vi "Decode Frames.vi"(8 "error in":errorcluster, 10 "data in":string, 11 "pending bytes":string) -> (0 "error out":errorcluster, 2 "decoded frames":T1[](array[typedef]), 3 "remaining bytes":string)   [LabVIEW 2015, in "Lengmur_socket.lvlib"]
uses:
  Lengmur_socket.lvlib
  Types/Decoded Frame.ctl
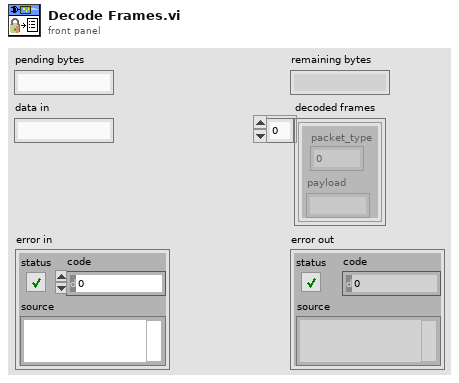
[diagram p1: front panel]
types:
  T1 = typedef "Lengmur_socket.lvlib/Decoded Frame.ctl" = cluster{"packet_type":u8, "payload":string}
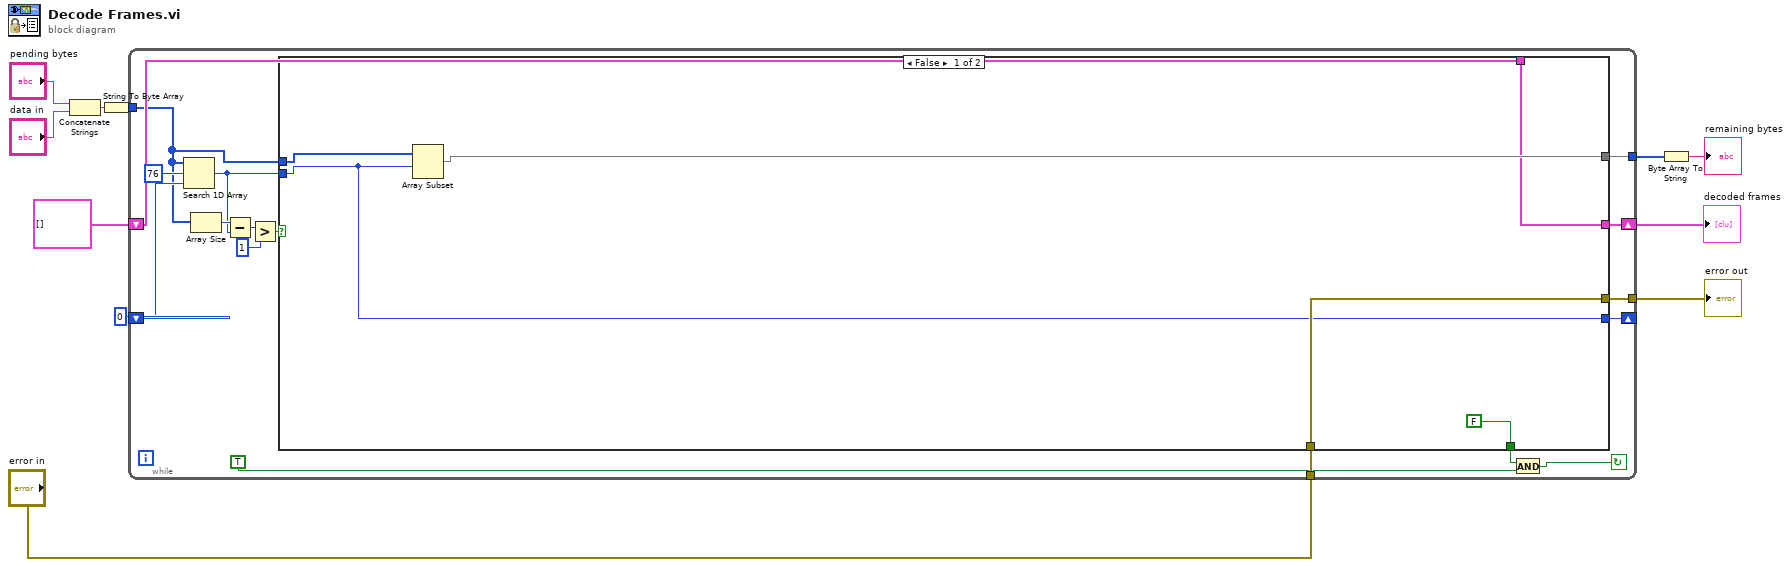
[diagram p0: block diagram]
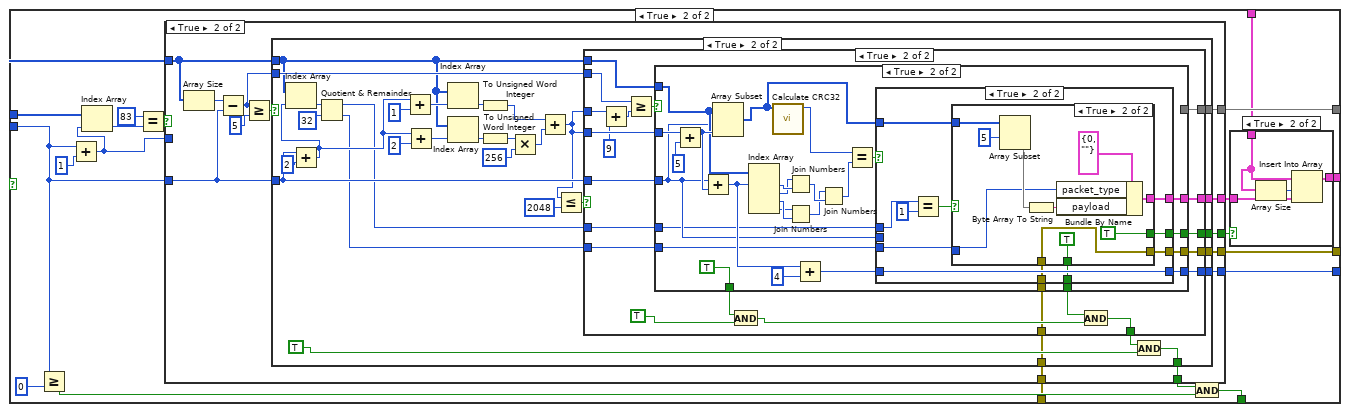
[diagram p2: hidden frame]
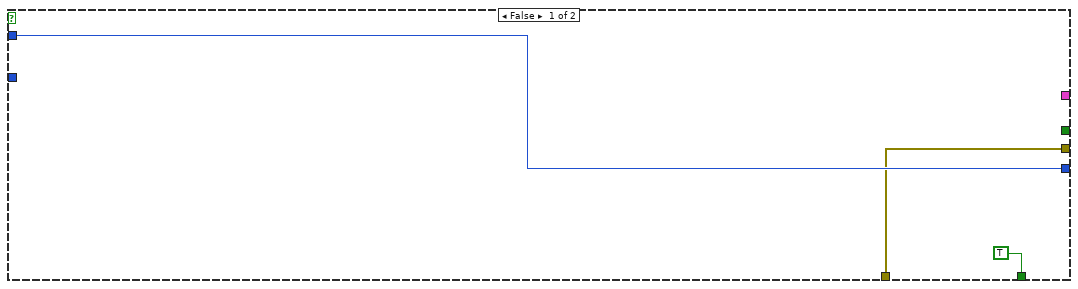
[diagram p3: hidden frame]
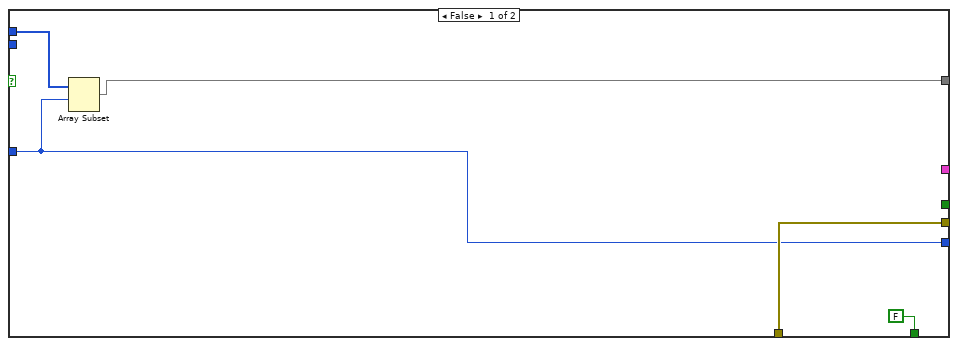
[diagram p4: hidden frame]
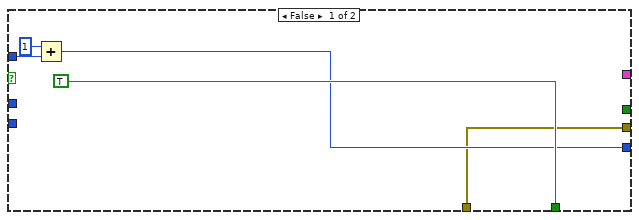
[diagram p5: hidden frame]
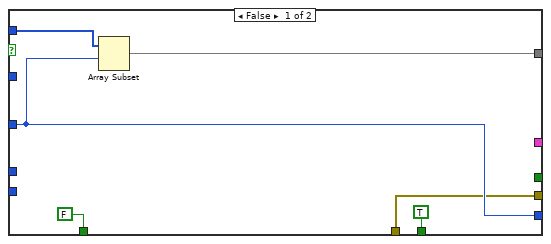
[diagram p6: hidden frame]
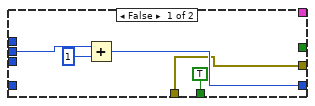
[diagram p7: hidden frame]
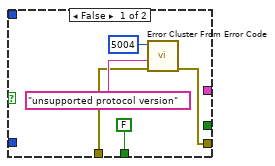
[diagram p8: hidden frame]
diagram:
  n1 = Concatenate Strings("pending bytes", "data in") -> (w9:string)
  n2 = String To Byte Array(string=w9) -> (unsigned byte array=w6:u8[])
  n3 = while {
    tunnel: w6 -> [w19]
    shift-right: [w26] -> _
    shift-left: 0 -> [w27]
    tunnel: [w25] -> w1
    tunnel: "error in" -> [w24]
    tunnel: [w23] -> w2
    shift-right: [w22] -> w4
    shift-left: T1[] [] ("decoded_frames") -> [w21]
    stop <- w13 continue-if-true
    n4 = Search 1D Array(1D array=w19, element=u8 76, start index (0)=w27) -> (index of element=w18:i32)
    n5 = Array Size(array=w19) -> (size(s)=w20:i32)
    n6 = Subtract(x=w20, y=w18) -> (x-y=w17:i32)
    n7 = Greater?(x=w17, y=1) -> (0:w15:bool)
    n8 = case shown="False" w15 {
      tunnel: [w31 w48] -> w26
      tunnel: [w33 w47] -> w25
      tunnel: w24 -> [w32 w45]
      tunnel: [w32 w44] -> w23
      tunnel: [w29 w40] -> w22
      tunnel: w21 -> [w29 w39]
      tunnel: w19 -> [w34 w37]
      tunnel: w18 -> [w31 w36]
      tunnel: [FALSE w35] -> w12
      frame False {
        n9 = Array Subset(array=w34, index=w31) -> (w33:u8[])  [unwired: 1 in]
      }
      frame True {
        n10 = Greater Or Equal?(x=w36, y=0) -> (x >= y?=w49:bool)
        n11 = Add(x=w36, y=u8 1) -> (x+y=w42:i32)
        n12 = Index Array(array=w37, index=w42) -> (element=w43:u8)
        n13 = Equal?(x=u8 83, y=w43) -> (x = y?=w52:bool)
        n14 = case shown="True" w52 {
          tunnel: [w56 w60] -> w48
          tunnel: w42 -> [w56 _]
          tunnel: w37 -> [_ w65]
          tunnel: w36 -> [_ w61]
          tunnel: [_ w66] -> w47
          tunnel: [TRUE w64] -> w46
          tunnel: w45 -> [w54 w63]
          tunnel: [w54 w62] -> w44
          tunnel: [_ w58] -> w41
          tunnel: [_ w57] -> w38
          frame False {
          }
          frame True {
            n15 = Array Size(array=w65) -> (size(s)=w69:i32)
            n16 = Subtract(x=w69, y=w61) -> (x-y=w59:i32)
            n17 = Greater Or Equal?(x=w59, y=5) -> (x >= y?=w67:bool)
            n18 = case shown="True" w67 {
              tunnel: [w70 w82] -> w66
              tunnel: w65 -> [w71 w83]
              tunnel: [FALSE w91] -> w64
              tunnel: w63 -> [w73 w78]
              tunnel: [w73 w77] -> w62
              tunnel: w61 -> [w72 w86]
              tunnel: [w72 w85] -> w60
              tunnel: w59 -> [_ w84]
              tunnel: [_ w80] -> w58
              tunnel: [_ w79] -> w57
              frame False {
                n19 = Array Subset(array=w71, index=w72) -> (w70:u8[])  [unwired: 1 in]
              }
              frame True {
                n20 = Add(x=w86, y=2) -> (x+y=w99:i32)
                n21 = Index Array(array=w83, index=w99) -> (element=w104:u8)
                n22 = Quotient & Remainder(x=w104, y=u8 32) -> (x-y*floor(x/y)=w76:u8, floor(x/y)=w75:u8)
                n23 = Add(x=w99, y=1) -> (x+y=w102:i32)
                n24 = Add(x=w99, y=2) -> (x+y=w100:i32)
                n25 = Index Array(array=w83, index=w102) -> (element=w96:u8)
                n26 = Index Array(array=w83, index=w100) -> (element=w97:u8)
                n27 = To Unsigned Word Integer(number=w96) -> (unsigned 16bit integer=w92:u16)
                n28 = To Unsigned Word Integer(number=w97) -> (unsigned 16bit integer=w95:u16)
                n29 = Multiply(x=w95, y=u16 256) -> (x*y=w93:u16)
                n30 = Add(x=w92, y=w93) -> (x+y=w81:u16)
                n31 = Less Or Equal?(x=w81, y=u16 2048) -> (x <= y?=w87:bool)
                n32 = case shown="True" w87 {
                  tunnel: [TRUE w115] -> w88
                  tunnel: w86 -> [w109 w126]
                  tunnel: [w107 w120] -> w85
                  tunnel: w81 -> [_ w129]
                  tunnel: w84 -> [_ w130]
                  tunnel: w83 -> [_ w127]
                  tunnel: [_ w125] -> w82
                  tunnel: w81 -> [_ w123]
                  tunnel: w75 -> [_ w119]
                  tunnel: [_ w118] -> w80
                  tunnel: [_ w117] -> w79
                  tunnel: w76 -> [_ w116]
                  tunnel: w78 -> [w106 w112]
                  tunnel: [w106 w111] -> w77
                  frame False {
                    n33 = Add(x=1, y=w109) -> (x+y=w107:i32)
                  }
                  frame True {
                    n34 = Add(x=w129, y=u16 9) -> (x+y=w122:u16)
                    n35 = Greater Or Equal?(x=w130, y=w122) -> (x >= y?=w128:bool)
                    n36 = case shown="True" w128 {
                      tunnel: w127 -> [w137 w161]
                      tunnel: w126 -> [w134 w144]
                      tunnel: [w136 _] -> w125
                      tunnel: [FALSE TRUE] -> w124
                      tunnel: w123 -> [_ w164]
                      tunnel: [w134 w146] -> w120
                      tunnel: w119 -> [_ w147]
                      tunnel: [_ w143] -> w118
                      tunnel: [_ w142] -> w117
                      tunnel: w116 -> [_ w141]
                      tunnel: [TRUE w140] -> w113
                      tunnel: w112 -> [w132 w139]
                      tunnel: [w132 w138] -> w111
                      frame False {
                        n37 = Array Subset(array=w137, index=w134) -> (w136:u8[])  [unwired: 1 in]
                      }
                      frame True {
                        n38 = Add(x=w164, y=u16 5) -> (x+y=w162:u16)
                        n39 = Add(x=w144, y=w162) -> (x+y=w151:i32)
                        n40 = Array Subset(array=w161, index=w144, length=w162) -> (w148:u8[])
                        n41 = Index Array(array=w161, index #1=w151) -> (element #1=w160:u8, element #2=w159:u8, element #3=w158:u8, element #4=w157:u8)  [unwired: 3 in]
                        n42 = call "Calculate CRC32.vi"("data bytes"=w148) -> ("crc32"=w153:u32)  [unwired: 9 in, 1 out]
                        n43 = Join Numbers(hi=w159, lo=w160) -> ((hi.lo)=w156:u16)
                        n44 = Join Numbers(hi=w157, lo=w158) -> ((hi.lo)=w155:u16)
                        n45 = Add(x=w151, y=4) -> (x+y=w145:i32)
                        n46 = Join Numbers(hi=w155, lo=w156) -> ((hi.lo)=w154:u32)
                        n47 = Equal?(x=w153, y=w154) -> (x = y?=w149:bool)
                        n48 = case shown="True" w149 {
                          tunnel: w148 -> [_ w180]
                          tunnel: w147 -> [_ w179]
                          tunnel: [w168 w178] -> w146
                          tunnel: w145 -> [_ w178]
                          tunnel: w144 -> [w169 _]
                          tunnel: [_ w177] -> w143
                          tunnel: [_ w176] -> w142
                          tunnel: w141 -> [_ w174]
                          tunnel: [TRUE w172] -> w140
                          tunnel: w139 -> [w165 w171]
                          tunnel: [w165 w170] -> w138
                          frame False {
                            n49 = Add(x=w169, y=1) -> (x+y=w168:i32)
                          }
                          frame True {
                            n50 = Equal?(x=w174, y=u8 1) -> (x = y?=w173:bool)
                            n51 = case shown="True" w173 {
                              tunnel: w180 -> [_ w195]
                              tunnel: w179 -> [_ w190]
                              tunnel: [_ TRUE] -> w177
                              tunnel: [_ w188] -> w176
                              tunnel: [FALSE TRUE] -> w172
                              tunnel: w171 -> [w182 w186]
                              tunnel: [w181 w186] -> w170
                              frame False {
                                n52 = call <vilib>:"Error Cluster From Error Code.vi"("error in (no error)"=w182, "error message (\"\")"="unsupported protocol version" ("error message (\"\")"), "error code (0)"=5004) -> ("error out"=w181:errorcluster)  [unwired: 6 in]
                              }
                              frame True {
                                n53 = Array Subset(array=w195, index=5) -> (w191:u8[])  [unwired: 1 in]
                                n54 = Byte Array To String(unsigned byte array=w191) -> (string=w192:string)
                                n55 = Bundle By Name(cluster=T1 {"packet_type"=0, "payload"=""} ("decoded_frame"), "packet_type"=w190, "payload"=w192) -> (w188:T1)
                              }
                            }
                          }
                        }
                      }
                    }
                    n56 = And(x=w124, y=TRUE) -> (x .and. y?=w114:bool)
                    n57 = And(x=w113, y=w114) -> (x .and. y?=w115:bool)
                  }
                }
                n58 = And(x=w88, y=TRUE) -> (x .and. y?=w91:bool)
              }
            }
          }
        }
        n59 = And(x=w46, y=w49) -> (x .and. y?=w35:bool)
        n60 = case shown="True" w41 {
          tunnel: [w196 w200] -> w40
          tunnel: w39 -> [w196 w197]
          tunnel: w38 -> [_ w199]
          frame False {
          }
          frame True {
            n61 = Array Size(array=w197) -> (size(s)=w198:i32)
            n62 = Insert Into Array(array=w197, index=w198, new element=w199) -> (w200:T1[])
          }
        }
      }
    }
    n63 = And(x=w12, y=TRUE) -> (x .and. y?=w13:bool)
  }
  "decoded frames" <- w4
  "error out" <- w2
  n64 = Byte Array To String(unsigned byte array=w1) -> (string=→"remaining bytes":string)
